vi "Update_admin_details.vi"(7 "Enum":enum16{"add", "update", "read", "remove"}(ring), 8 "error in (no error)":errorcluster, 10 "string":string, 11 "User":string) -> (0 "error out":errorcluster, 3 "Status":bool)   [LabVIEW 2021]
panel:
  out "standard output":string
  out "standard error":string
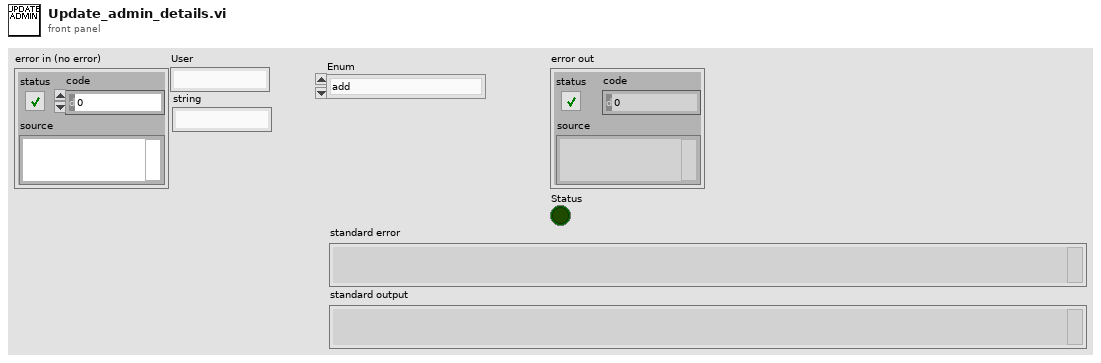
[diagram p1: front panel]
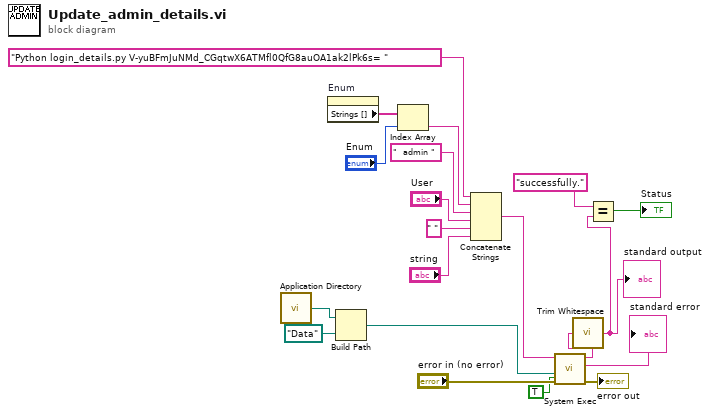
[diagram p0: block diagram]
diagram:
  n1 = call <vilib>:"Application Directory.vi"() -> ("Application Directory"=w1:path)
  n2 = property on="Enum" class="Enum (strict)"() -> ("Strings []"=w9:string[])  [unwired: 2 in, 2 out]
  n3 = Build Path(base path=w1, name or relative path=path "Data") -> (appended path=w15:path)
  n4 = Index Array(array=w9, index="Enum") -> (element=w7:string)
  n5 = Concatenate Strings("Python login_details.py V-yuBFmJuNMd_CGqtwX6ATMfl0QfG8auOA1ak2lPk6s= " ("string"), w7, "  admin ", "User", " " ("string"), "string") -> (w17:string)
  n6 = call <vilib>:"System Exec.vi"("run minimized? (F)"=TRUE, "error in (no error)"="error in (no error)", "working directory"=w15, "command line"=w17) -> ("error out"=→"error out":errorcluster, "standard error"=→"standard error":string, "standard output"=w4:string)  [unwired: 4 in, 1 out]
  n7 = call <vilib>:"Trim Whitespace.vi"("string"=w4) -> ("trimmed string"=w3:string)  [unwired: 1 in]
  "standard output" <- w3
  n8 = Equal?(x="successfully.", y=w3) -> (x = y?=→"Status":bool)
